vi "Write Mast Speed.vi"(8 "error in (no error)":errorcluster, 10 "Speed (1~8)":i32=1 min=1 max=8, 11 "CO3000 in":refnum<class "CO3000.lvclass">) -> (0 "error out":errorcluster, 3 "CO3000 out":refnum<class "CO3000.lvclass">)   [LabVIEW 2023, in "Turn Table and Mast.lvlib" / "CO3000.lvclass"]
uses:
  CO3000.lvclass
  CO3000.lvclass/CO3000.ctl
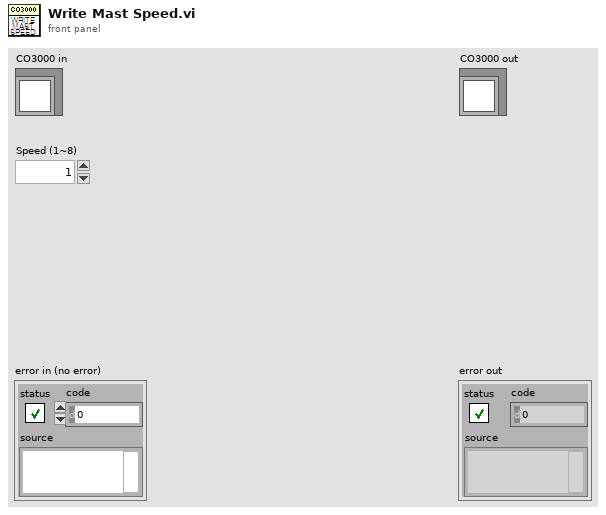
[diagram p1: front panel]
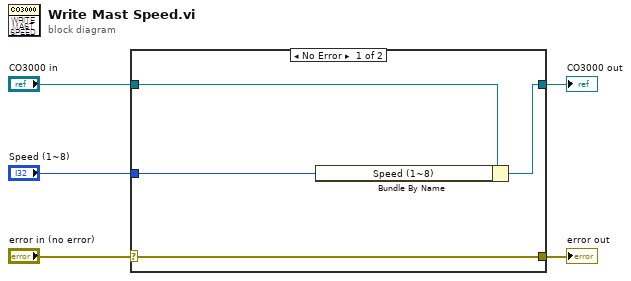
[diagram p0: block diagram]
diagram:
  n1 = case shown="No Error" "error in (no error)" {
    selector: "error in (no error)" -> [w9 w10]
    tunnel: [w9 w10] -> w4
    tunnel: [w7 w11] -> w2
    tunnel: "CO3000 in" -> [w8 w11]
    tunnel: "Speed (1~8)" -> [w6 _]
    frame No Error {
      n2 = Bundle By Name(cluster=w8, "Speed (1~8)"=w6) -> (w7:refnum<class "CO3000.lvclass">)
    }
    frame Error {
    }
  }
  "error out" <- w4
  "CO3000 out" <- w2
